vi "CIVI Set Mode Example.vi"() -> ()   [LabVIEW 2026]
panel:
  out "SCPI Error Code":i32
  in  "Mode Setpint":string
  out "Operation Complete":string
  out "S Meter (raw)":i32
  out "Mode":string
  out "error out":errorcluster
  out "Frequency (Hz)":i32
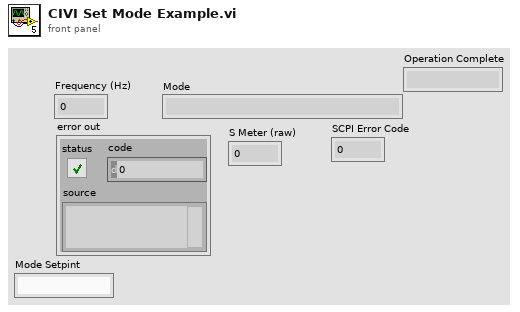
[diagram p1: front panel]
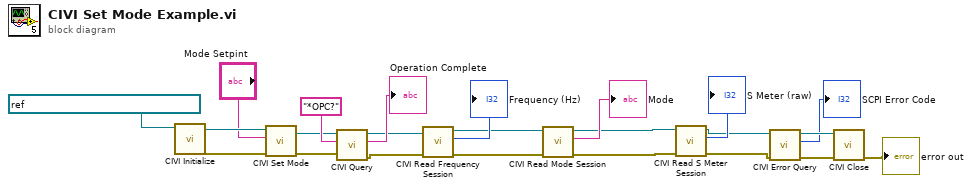
[diagram p0: block diagram]
diagram:
  n1 = call "CIVI Initialize.vi"("VISA Resource Name"=refnum<visa-resource-name> "TCPIP0::127.0.0.1::5025::SOCKET") -> ("error out"=w8:errorcluster, "VISA Session out"=w9:refnum<visa-resource-name>)  [unwired: 9 in]
  n2 = call "CIVI Set Mode.vi"("error in (no error)"=w8, "Mode"="Mode Setpint", "VISA Refnum in"=w9) -> ("error out"=w7:errorcluster, "VISA Refnum out"=w10:refnum<visa-resource-name>)  [unwired: 7 in]
  n3 = call "CIVI Query.vi"("error in"=w7, "write buffer"="*OPC?", "VISA Session in"=w10) -> ("error out"=w11:errorcluster, "read buffer"=→"Operation Complete":string, "VISA Session out"=w12:refnum<visa-resource-name>)  [unwired: 6 in]
  n4 = call "CIVI Read Frequency Session.vi"("error in"=w11, "VISA Session in"=w12) -> ("error out"=w19:errorcluster, "Frequency (Hz)"=→"Frequency (Hz)":i32, "VISA Session out"=w20:refnum<visa-resource-name>)  [unwired: 7 in]
  n5 = call "CIVI Read Mode Session.vi"("error in"=w19, "VISA Session in"=w20) -> ("error out"=w16:errorcluster, "Mode"=→"Mode":string, "VISA Session out"=w17:refnum<visa-resource-name>)  [unwired: 7 in]
  n6 = call "CIVI Read S Meter Session.vi"("error in"=w16, "VISA Session in"=w17) -> ("error out"=w2:errorcluster, "S Meter (raw)"=→"S Meter (raw)":i32, "VISA Session out"=w3:refnum<visa-resource-name>)  [unwired: 7 in]
  n7 = call "CIVI Error Query.vi"("error in"=w2, "VISA Session in"=w3) -> ("error out"=w5:errorcluster, "SCPI Error Code"=→"SCPI Error Code":i32, "VISA Session out"=w4:refnum<visa-resource-name>)  [unwired: 7 in]
  n8 = call "CIVI Close.vi"("error in"=w5, "VISA Session in"=w4) -> ("error out"=→"error out":errorcluster)  [unwired: 9 in]
